vi "VM Spy - set probe window position.vi"(6 "error in":errorcluster, 9 "refnum":refnum<vi>) -> (0 "error out":errorcluster, 3 "dup refnum":refnum<vi>)   [LabVIEW 2021]
doc: "::: CalcExpress Toolkit :::\nCopyright (c) 2000-2026 Konstantin Shifershteyn. All rights reserved."
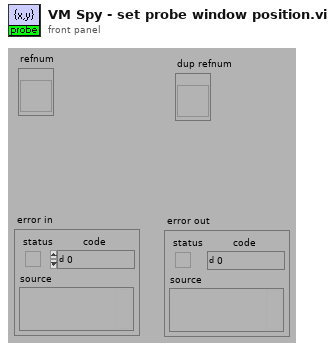
[diagram p1: front panel]
types:
  T1 = typedef "LVRectTypeDef.ctl" = cluster{"Left":i16, "Top":i16, "Right":i16, "Bottom":i16}
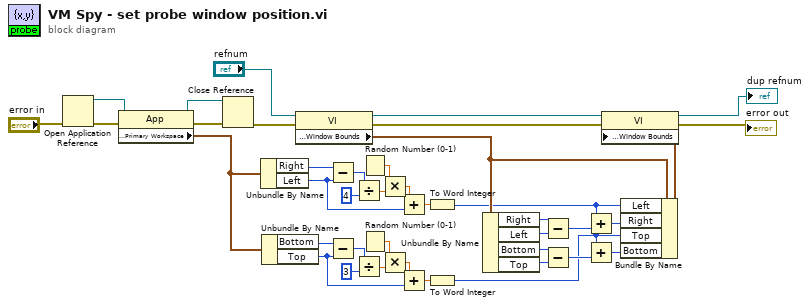
[diagram p0: block diagram]
diagram:
  n1 = Open Application Reference(8:"error in") -> (0:w31:errorcluster, 3:w39:refnum<vi>)  [unwired: 3 in]
  n2 = property class="App"(reference=w39, error in=w31) -> (reference out=w38:refnum<vi>, error out=w30:errorcluster, "Display:Primary Workspace"=w8:T1)
  n3 = Close Reference(reference=w38, error in (no error)=w30) -> (error out=w29:errorcluster)
  n4 = Unbundle By Name(w8) -> ("Right"=w24:i16, "Left"=w20:i16)
  n5 = Unbundle By Name(w8) -> ("Bottom"=w9:i16, "Top"=w13:i16)
  n6 = property class="VI"(reference="refnum", error in=w29) -> (reference out=w33:refnum<vi>, error out=w27:errorcluster, "Front Panel Window:Window Bounds"=w32:T1)
  n7 = Subtract(x=w24, y=w20) -> (x-y=w23:i16)
  n8 = Subtract(x=w9, y=w13) -> (x-y=w10:i16)
  n9 = Divide(x=w23, y=i16 4) -> (x/y=w18:dbl)
  n10 = Divide(x=w10, y=i16 3) -> (x/y=w15:dbl)
  n11 = Random Number (0-1)() -> (number: 0 to 1=w17:dbl)
  n12 = Random Number (0-1)() -> (number: 0 to 1=w16:dbl)
  n13 = Multiply(x=w17, y=w18) -> (x*y=w21:dbl)
  n14 = Multiply(x=w16, y=w15) -> (x*y=w12:dbl)
  n15 = Add(x=w21, y=w20) -> (x+y=w19:dbl)
  n16 = Add(x=w12, y=w13) -> (x+y=w14:dbl)
  n17 = To Word Integer(number=w19) -> (16bit integer=w2:i16)
  n18 = To Word Integer(number=w14) -> (16bit integer=w1:i16)
  n19 = Unbundle By Name(w32) -> ("Right"=w37:i16, "Left"=w36:i16, "Bottom"=w35:i16, "Top"=w34:i16)
  n20 = Subtract(x=w37, y=w36) -> (x-y=w3:i16)
  n21 = Subtract(x=w35, y=w34) -> (x-y=w4:i16)
  n22 = Add(x=w2, y=w3) -> (x+y=w6:i16)
  n23 = Add(x=w1, y=w4) -> (x+y=w5:i16)
  n24 = Bundle By Name(cluster=w32, "Left"=w2, "Right"=w6, "Top"=w1, "Bottom"=w5) -> (w7:T1)
  n25 = property class="VI"(reference=w33, error in=w27, "Front Panel Window:Window Bounds"=w7) -> (reference out=→"dup refnum":refnum<vi>, error out=→"error out":errorcluster)
